vi "labview-quick-asset.vi"   [LabVIEW 2020]
uses:
  Nominal Client/Nominal Client.lvclass/Nominal Client.ctl
  User/User.lvclass
  Nominal Client/Nominal Client.lvclass
  nominal types/workspace/workspace.lvclass
  submodules/reqwest-labview/lv-src/reqwest/reqwest.lvclass
  e79185ee-863a-4b48-b269-365b27d9e424.vi
  asset/asset.lvclass
  Nominal Client/asset.get.vi
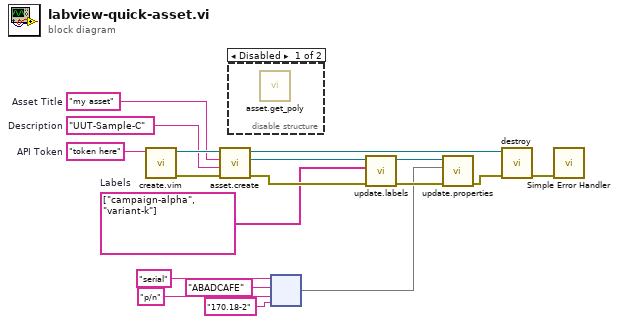
[diagram p0: block diagram]
diagram:
  w6 = string[] ["campaign-alpha", "variant-k"]  # Labels
  w12 = "UUT-Sample-C"  # Description
  w13 = "token here"  # API Token
  w14 = "my asset"  # Asset Title
  n1 = call "create.vim"("API Token (string or path)"=w13) -> ("error out"=w17:errorcluster, "Nominal Client"=w18:refnum<class "Nominal Client.lvclass">)  [unwired: 8 in, 1 out]
  n2 = call "asset.create.vi"("error in"=w17, "Description"=w12, "Title"=w14, "Nominal Client in"=w18) -> ("error out"=w10:errorcluster, "asset"=w11:refnum<class "asset.lvclass">, "Nominal Client out"=w16:refnum<class "Nominal Client.lvclass">)  [unwired: 5 in]
  n3 = disable-structure shown="Disabled" {
    frame Disabled {
      n4 = call-poly "asset.get_poly.vi"() -> ()  [unwired: 9 in, 3 out]
    }
    frame Enabled {
    }
  }
  n5 = node("serial", "ABADCAFE", "p/n", "170.18-2") -> (w1:map{string, string})
  n6 = call "update.labels.vi"("error in"=w10, "Labels"=w6, "asset in"=w11) -> ("error out"=w8:errorcluster, "asset out"=w9:refnum<class "asset.lvclass">)  [unwired: 7 in]
  n7 = call "update.properties.vi"("error in"=w8, "Properties"=w1, "asset in"=w9) -> ("error out"=w7:errorcluster)  [unwired: 7 in, 1 out]
  n8 = call "destroy.vi"("error in"=w7, "Nominal Client"=w16) -> ("error out"=w15:errorcluster)  [unwired: 9 in]
  n9 = call <vilib>:"Simple Error Handler.vi"("error in (no error)"=w15) -> ()  [unwired: 4 in, 5 out]
